vi "measure PSD Marker Value Type.vi"(8 "error in (no error)":errorcluster, 11 "SA Measurement in":refnum<class "SA Measurement.lvclass">) -> (0 "error out":errorcluster, 3 "SA Measurement out":refnum<class "SA Measurement.lvclass">)   [LabVIEW 2023, in "Spectrum Analyzer.lvlib" / "SA Measurement.lvclass"]
uses:
  SA Measurement.lvclass
  SA Measurement.lvclass/SA Measurement.ctl
  TYPE DEFINITION/Keysight 9020A/TYPE Measurement Preset.ctl
  Spectrum Analyzer.lvlib
  TYPE DEFINITION/TYPE RBW and VBW Select.ctl
  Interface_Spectrum/Interface_Spectrum.lvclass
  TYPE DEFINITION/TYPE Marker Peak Search Type.ctl
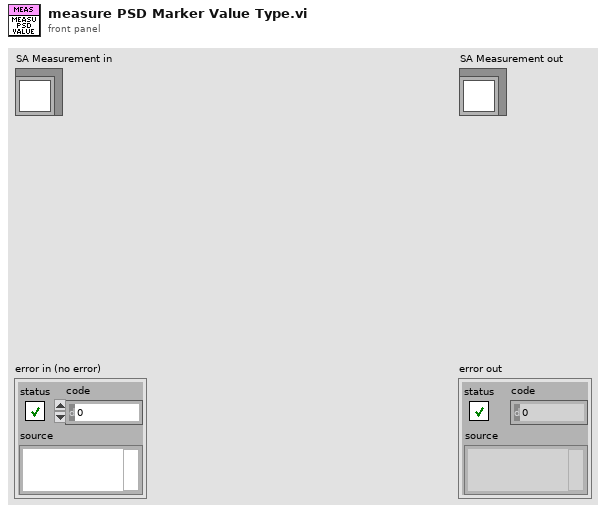
[diagram p1: front panel]
types:
  T1 = typedef "Spectrum Analyzer.lvlib/TYPE Marker Peak Search Type.ctl" = enum16{"Max", "Next Peak", "Max - Auto"}
  T2 = typedef "Spectrum Analyzer.lvlib/TYPE RBW and VBW Select.ctl" = enum16{"Res BW", "Video BW"}
  T3 = typedef "Spectrum Analyzer.lvlib/TYPE Measurement Preset.ctl" = enum16{"Sweep SA Mode", "Channel Power", "Occupied BW", "ACP", "Spurious Emission", "Spurious Emission Mask", "Burst Power (Transmit Power)"}
  T4 = typedef "Spectrum Analyzer.lvlib/TYPE Y-axis Unit.ctl" = enum16{"dBm", "dBmV", "dBuV", "dBpW", "Volt", "Ampere", "Watt"}
  T5 = typedef "Spectrum Analyzer.lvlib/TYPE Reference Level and Atten Param.ctl" = cluster{"Reference Level":dbl, "Atten":i32, "Atten Auto?":bool, "Reference Level Offset":dbl}
  T6 = typedef "Spectrum Analyzer.lvlib/TYPE Display Trace Mode Select.ctl" = enum16{"Clear Write", "Max Hold", "Min Hold", "Average", "View"}
  T7 = typedef "Spectrum Analyzer.lvlib/TYPE Detect Mode Select.ctl" = enum16{"Det Auto (Normal)", "Auto Peak", "Positive Peak", "Negative Peak", "Sample", "RMS", "Average", "Quasipeak", "CISPR Average", "RMS Average"}
  T8 = cluster{"Trace Mode":T6, "Detector Type":T7, "Detect Auto?":bool}[]
  T9 = typedef "Spectrum Analyzer.lvlib/TYPE Average Mode Select.ctl" = enum16{"Linear(Voltage Avg)", "Video(Log)", "Power"}
  T10 = typedef "Spectrum Analyzer.lvlib/TYPE Marker Value.ctl" = cluster{"X-axis":dbl, "Y-axis":dbl}
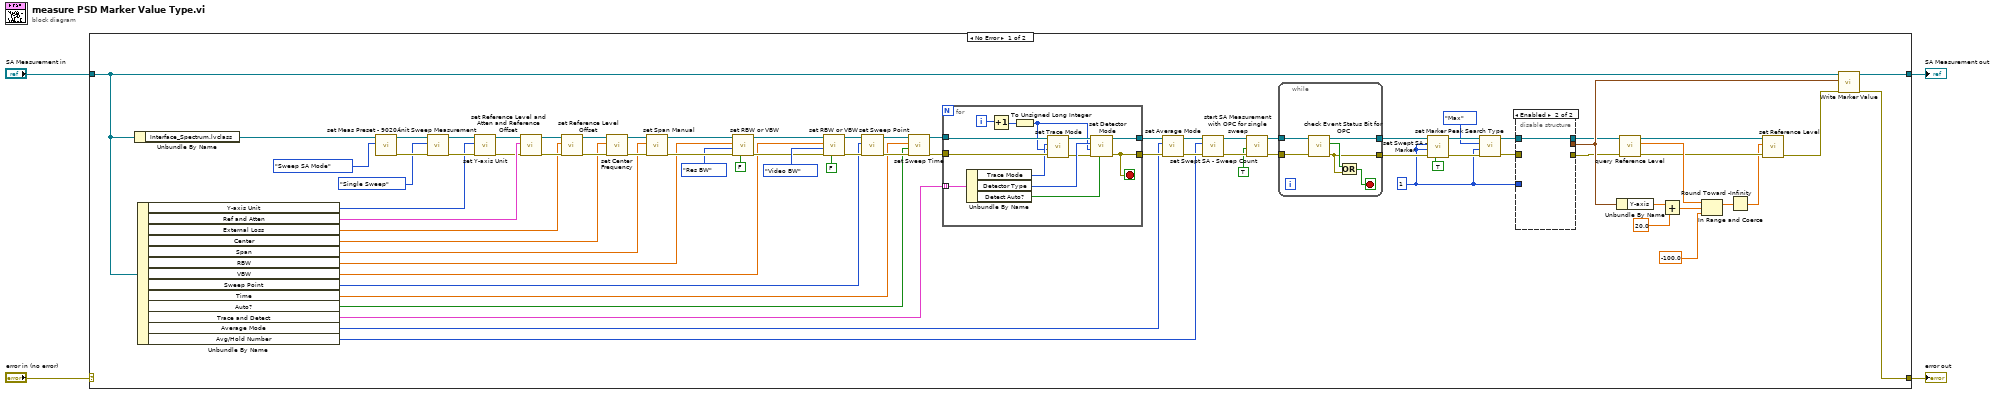
[diagram p0: block diagram]
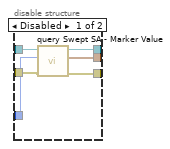
[diagram p2: hidden frame]
diagram:
  n1 = case shown="No Error" "error in (no error)" {
    selector: "error in (no error)" -> [_ w108]
    tunnel: [w19 w108] -> w3
    tunnel: [w20 w107] -> w1
    tunnel: "SA Measurement in" -> [w18 w107]
    frame No Error {
      w21 = 1 ("Index")
      n2 = Unbundle By Name(w18) -> ("Interface_Spectrum.lvclass"=w80:refnum<class "Interface_Spectrum.lvclass">)
      n3 = Unbundle By Name(w18) -> ("Y-axis Unit"=w51:T4, "Ref and Atten"=w75:T5, "External Loss"=w72:dbl, "Center"=w69:dbl, "Span"=w66:dbl, "RBW"=w63:dbl, "VBW"=w56:dbl, "Sweep Point"=w48:u32, "Time"=w45:dbl, "Auto?"=w44:bool, "Trace and Detect"=w41:T8, "Average Mode"=w38:T9, "Avg/Hold Number"=w35:u32)
      n4 = call-dynamic "set Meas Preset - 9020A.vi"("Measurement Preset"=TYPE_Measurement_Preset."Sweep SA Mode", "Interface_Spectrum in"=w80) -> ("error out"=w77:errorcluster, "Interface_Spectrum out"=w78:refnum<class "Interface_Spectrum.lvclass">)  [unwired: 8 in]
      n5 = call-dynamic "init Sweep Measurement.vi"("error in (no error)"=w77, "Sweep Measurement Mode"=enum16{"Single Sweep", "Continuous Sweep"}."Single Sweep", "Interface_Spectrum in"=w78) -> ("error out"=w54:errorcluster, "Interface_Spectrum out"=w55:refnum<class "Interface_Spectrum.lvclass">)  [unwired: 7 in]
      n6 = call-dynamic "set Y-axis Unit.vi"("error in (no error)"=w54, "Y-axis Unit"=w51, "Interface_Spectrum in"=w55) -> ("error out"=w52:errorcluster, "Interface_Spectrum out"=w53:refnum<class "Interface_Spectrum.lvclass">)  [unwired: 7 in]
      n7 = call-dynamic "set Reference Level and Atten and Reference Offset.vi"("error in (no error)"=w52, "Reference Level, Atten, Reference Offset"=w75, "Interface_Spectrum in"=w53) -> ("error out"=w73:errorcluster, "Interface_Spectrum out"=w74:refnum<class "Interface_Spectrum.lvclass">)  [unwired: 7 in]
      n8 = call-dynamic "set Reference Level Offset.vi"("error in (no error)"=w73, "Reference Level Offset"=w72, "Interface_Spectrum in"=w74) -> ("error out"=w70:errorcluster, "Interface_Spectrum out"=w71:refnum<class "Interface_Spectrum.lvclass">)  [unwired: 7 in]
      n9 = call-dynamic "set Center Frequency.vi"("error in (no error)"=w70, "Center Frequency (Hz)"=w69, "Interface_Spectrum in"=w71) -> ("error out"=w67:errorcluster, "Interface_Spectrum out"=w68:refnum<class "Interface_Spectrum.lvclass">)  [unwired: 7 in]
      n10 = call-dynamic "set Span Manual.vi"("error in (no error)"=w67, "Span (Hz)"=w66, "Interface_Spectrum in"=w68) -> ("error out"=w64:errorcluster, "Interface_Spectrum out"=w65:refnum<class "Interface_Spectrum.lvclass">)  [unwired: 7 in]
      n11 = call-dynamic "set RBW or VBW.vi"("BW Auto?"=FALSE, "error in (no error)"=w64, "BW Type"=TYPE_RBW_and_VBW_Select."Res BW", "BW Value (Hz)"=w63, "Interface_Spectrum in"=w65) -> ("error out"=w57:errorcluster, "Interface_Spectrum out"=w58:refnum<class "Interface_Spectrum.lvclass">)  [unwired: 5 in]
      n12 = call-dynamic "set RBW or VBW.vi"("BW Auto?"=FALSE, "error in (no error)"=w57, "BW Type"=TYPE_RBW_and_VBW_Select."Video BW", "BW Value (Hz)"=w56, "Interface_Spectrum in"=w58) -> ("error out"=w49:errorcluster, "Interface_Spectrum out"=w50:refnum<class "Interface_Spectrum.lvclass">)  [unwired: 5 in]
      n13 = call-dynamic "set Sweep Point.vi"("error in (no error)"=w49, "Sweep Point"=w48, "Interface_Spectrum in"=w50) -> ("error out"=w46:errorcluster, "Interface_Spectrum out"=w47:refnum<class "Interface_Spectrum.lvclass">)  [unwired: 7 in]
      n14 = call-dynamic "set Sweep Time.vi"("error in (no error)"=w46, "Sweep Time Auto?"=w44, "Sweep Time(sec)"=w45, "Interface_Spectrum in"=w47) -> ("error out"=w42:errorcluster, "Interface_Spectrum out"=w43:refnum<class "Interface_Spectrum.lvclass">)  [unwired: 6 in]
      n15 = for {
        tunnel: w43 -> [w105]
        tunnel: w42 -> [w104]
        tunnel: w41 -> [w106] mode=indexing
        tunnel: [w94] -> w39
        tunnel: [w95] -> w40
        i -> [w103]
        stop <- w94 stop-if-true
        n16 = Unbundle By Name(w106) -> ("Trace Mode"=w101:T6, "Detector Type"=w99:T7, "Detect Auto?"=w96:bool)
        n17 = Increment(x=w103) -> (x+1=w102:i32)
        n18 = To Unsigned Long Integer(number=w102) -> (unsigned 32bit integer=w97:u32)
        n19 = call-dynamic "set Trace Mode.vi"("error in (no error)"=w104, "Trace Index"=w97, "Trace Mode"=w101, "Interface_Spectrum in"=w105) -> ("error out"=w98:errorcluster, "Interface_Spectrum out"=w100:refnum<class "Interface_Spectrum.lvclass">)  [unwired: 6 in]
        n20 = call-dynamic "set Detector Mode.vi"("Detect Auto?"=w96, "error in (no error)"=w98, "Trace Index"=w97, "Detector Type"=w99, "Interface_Spectrum in"=w100) -> ("error out"=w94:errorcluster, "Interface_Spectrum out"=w95:refnum<class "Interface_Spectrum.lvclass">)  [unwired: 5 in]
      }
      n21 = call-dynamic "set Average Mode.vi"("error in (no error)"=w39, "Average Mode"=w38, "Interface_Spectrum in"=w40) -> ("error out"=w36:errorcluster, "Interface_Spectrum out"=w37:refnum<class "Interface_Spectrum.lvclass">)  [unwired: 7 in]
      n22 = call-dynamic "set Swept SA - Sweep Count.vi"("error in (no error)"=w36, "Sweep Count"=w35, "Interface_Spectrum in"=w37) -> ("error out"=w33:errorcluster, "Interface_Spectrum out"=w34:refnum<class "Interface_Spectrum.lvclass">)  [unwired: 7 in]
      n23 = call-dynamic "start SA Measurement with OPC for single sweep.vi"("error in (no error)"=w33, "with OPC?"=TRUE, "Interface_Spectrum in"=w34) -> ("error out"=w30:errorcluster, "Interface_Spectrum out"=w31:refnum<class "Interface_Spectrum.lvclass">)  [unwired: 7 in]
      n24 = while {
        tunnel: w31 -> [w93]
        tunnel: w30 -> [w92]
        tunnel: [w89] -> w28
        tunnel: [w88] -> w29
        stop <- w90 stop-if-true
        n25 = call-dynamic "check Event Status Bit for OPC.vi"("error in (no error)"=w92, "Interface_Spectrum in"=w93) -> ("error out"=w89:errorcluster, "OPC Bit Changed?"=w91:bool, "Interface_Spectrum out"=w88:refnum<class "Interface_Spectrum.lvclass">)  [unwired: 7 in]
        n26 = Or(x=w91, y=w89) -> (x .or. y?=w90:bool)
      }
      n27 = call-dynamic "set Swept SA - Marker.vi"("On?"=TRUE, "error in (no error)"=w28, "trace"=w21, "Index"=w21, "Interface_Spectrum in"=w29) -> ("error out"=w25:errorcluster, "Interface_Spectrum out"=w26:refnum<class "Interface_Spectrum.lvclass">)  [unwired: 5 in]
      n28 = call-dynamic "set Marker Peak Search Type.vi"("error in (no error)"=w25, "Marker Index"=w21, "Peak Search Type"=TYPE_Marker_Peak_Search_Type."Max", "Interface_Spectrum in"=w26) -> ("error out"=w22:errorcluster, "Interface_Spectrum out"=w23:refnum<class "Interface_Spectrum.lvclass">)  [unwired: 6 in]
      n29 = disable-structure shown="Enabled" {
        disable-tunnel: w23 -> [w86 w87]
        disable-tunnel: w22 -> [w85 _]
        disable-tunnel: w21 -> [w84 _]
        disable-tunnel: [w83 _] -> w15
        disable-tunnel: [w82 w87] -> w13
        disable-tunnel: [w81 _] -> w12
        frame Disabled {
          n30 = call-dynamic "query Swept SA - Marker Value.vi"("error in (no error)"=w85, "Marker Index"=w84, "Interface_Spectrum in"=w86) -> ("error out"=w81:errorcluster, "Marker Value"=w83:T10, "Interface_Spectrum out"=w82:refnum<class "Interface_Spectrum.lvclass">)  [unwired: 6 in]
        }
        frame Enabled {
        }
      }
      n31 = Unbundle By Name(w15) -> ("Y-axis"=w17:dbl)
      n32 = call-dynamic "query Reference Level.vi"("error in (no error)"=w12, "Interface_Spectrum in"=w13) -> ("error out"=w7:errorcluster, "Ref Level"=w10:dbl, "Interface_Spectrum out"=w11:refnum<class "Interface_Spectrum.lvclass">)  [unwired: 7 in]
      n33 = Add(x=w17, y=20.0) -> (x+y=w9:dbl)
      n34 = In Range and Coerce(upper limit=w10, x=w9, lower limit=-100.0) -> (coerced(x)=w6:dbl)  [unwired: 1 out]
      n35 = Round Toward -Infinity(1:w6) -> (0:w5:dbl)
      n36 = call-dynamic "set Reference Level.vi"("error in (no error)"=w7, "Reference Level"=w5, "Interface_Spectrum in"=w11) -> ("error out"=w14:errorcluster)  [unwired: 7 in, 1 out]
      n37 = call "Write Marker Value.vi"("error in (no error)"=w14, "Marker Value"=w15, "SA Measurement in"=w18) -> ("error out"=w19:errorcluster, "SA Measurement out"=w20:refnum<class "SA Measurement.lvclass">)  [unwired: 7 in]
    }
    frame Error {
    }
  }
  "error out" <- w3
  "SA Measurement out" <- w1
